vi "GDSIconEditor_SplitNameInRows.vi"(9 "FileNameFilter":T1, 11 "name":string) -> (3 "result string":string)   [LabVIEW 2020]
uses:
  GDSIconEditor_FileNameFilter.ctl
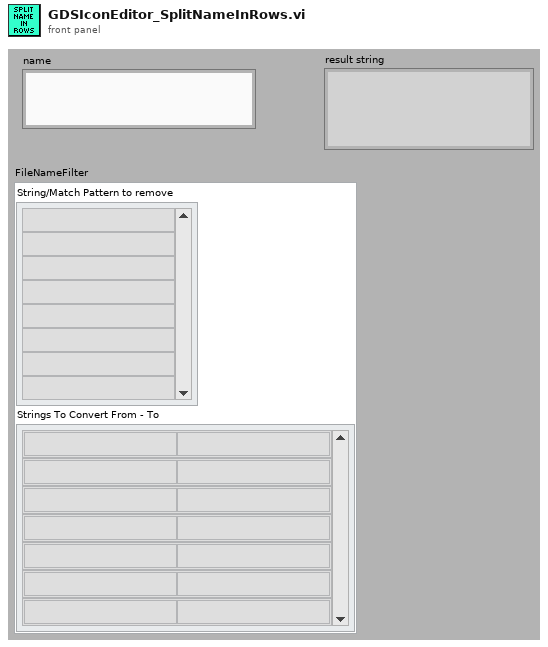
[diagram p1: front panel]
types:
  T1 = typedef "GDSIconEditor_FileNameFilter.ctl" = cluster{"String/Match Pattern to remove":string[], "Strings To Convert From - To":cluster{"From":string, "To":string}[]}
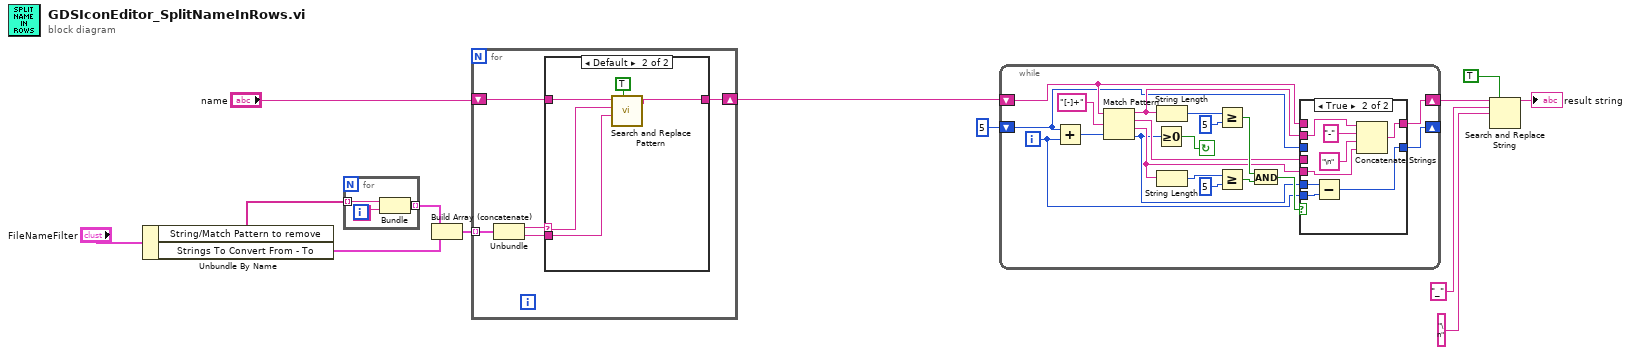
[diagram p0: block diagram]
diagram:
  n1 = Unbundle By Name("FileNameFilter") -> ("String/Match Pattern to remove"=w5:string[], "Strings To Convert From - To"=w3:cluster{"From":string, "To":string}[])
  n2 = for {
    tunnel: w5 -> [w16] mode=indexing
    tunnel: [w14] -> w4 mode=indexing
    n3 = Bundle("String"=w16, "") -> (w14:cluster{"String":string, string})  [unwired: 1 in]
  }
  n4 = Build Array (concatenate)(w4, w3) -> (w2:cluster{"From":string, "To":string}[])
  n5 = for {
    shift-right: [w20] -> w1
    shift-left: "name" -> [w21]
    tunnel: w2 -> [w19] mode=indexing
    n6 = Unbundle(w19) -> ("From"=w18:string, "To"=w17:string)
    n7 = case shown="Default" w18 {
      selector: w18 -> [_ w24]
      tunnel: w21 -> [w22 w27]
      tunnel: [w22 w26] -> w20
      tunnel: w17 -> [_ w23]
      frame "" {
      }
      frame Default {
        n8 = call <vilib>:"Search and Replace Pattern.vi"("string"=w27, "regular expression (\"\")"=w24, "replace string (\"\")"=w23, "replace all? (F)"=TRUE) -> ("result string"=w26:string)  [unwired: 1 in, 1 out]
      }
    }
  }
  n9 = while {
    shift-right: [w38] -> w8
    shift-left: w1 -> [w37]
    shift-right: [w31] -> _
    shift-left: 5 -> [w30]
    i -> [w32]
    stop <- w28 continue-if-true
    n10 = Add(x=w30, y=w32) -> (x+y=w36:i32)
    n11 = Match Pattern(string=w37, regular expression="[-]+", offset (0)=w36) -> (before substring=w35:string, match substring=w34:string, after substring=w33:string, offset past match=w29:i32)
    n12 = Greater Or Equal To 0?(x=w29) -> (x >= 0?=w28:bool)
    n13 = String Length(string=w35) -> (length=w45:i32)
    n14 = String Length(string=w33) -> (length=w43:i32)
    n15 = Greater Or Equal?(x=w45, y=5) -> (x >= y?=w41:bool)
    n16 = Greater Or Equal?(x=w43, y=5) -> (x >= y?=w40:bool)
    n17 = And(x=w41, y=w40) -> (x .and. y?=w39:bool)
    n18 = case shown="True" w39 {
      tunnel: w37 -> [w48 _]
      tunnel: [w48 w53] -> w38
      tunnel: w35 -> [_ w56]
      tunnel: w34 -> [_ _]
      tunnel: w33 -> [_ w54]
      tunnel: w29 -> [_ w52]
      tunnel: w32 -> [_ w51]
      tunnel: [w47 w50] -> w31
      tunnel: w30 -> [w47 _]
      frame False {
      }
      frame True {
        n19 = Subtract(x=w52, y=w51) -> (x-y=w50:i32)
        n20 = Concatenate Strings(w56, "-" ("string"), "\n" ("string"), w54) -> (w53:string)
      }
    }
  }
  n21 = Search and Replace String(replace all?=TRUE ("replace all? (F)"), input string=w8, search string="_", replace string="\n" ("replace string (\"\")")) -> (result string=→"result string":string)  [unwired: 4 in, 3 out]
